vi "Create New File.vi"(8 "error in (no error)":errorcluster, 11 "file handler in":refnum<class "File Handler.lvclass">) -> (0 "error out":errorcluster, 3 "file handler out":refnum<class "File Handler.lvclass">)   [LabVIEW 2018, in "GLog.lvlib" / "File Handler.lvclass"]
uses:
  File Handler.lvclass
  File Handler.lvclass/File Handler.ctl
  Send Update Event.vi
  RolloverTrigger/RolloverTrigger.lvclass
panel:
  # "Connector Pane"
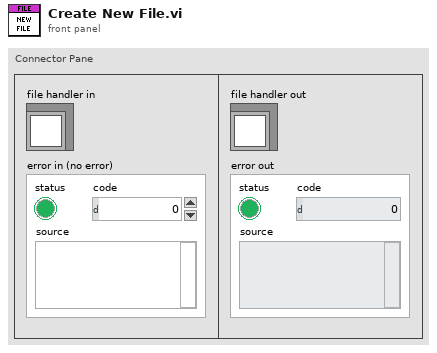
[diagram p1: front panel]
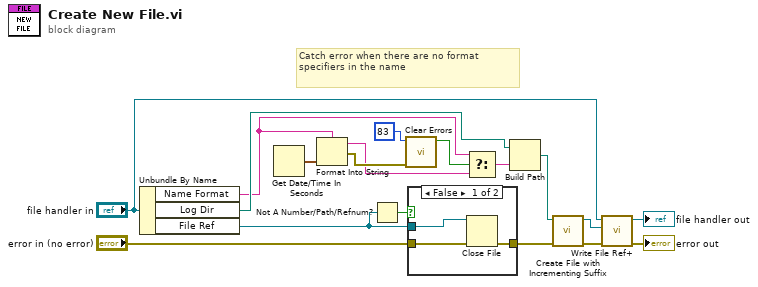
[diagram p0: block diagram]
diagram:
  # "Catch error when there are no format specifiers in the name"
  n1 = Unbundle By Name("file handler in") -> ("Name Format"=w3:string, "Log Dir"=w17:path, "File Ref"=w13:refnum<file>)
  n2 = Get Date/Time In Seconds() -> (seconds since 1Jan1904=w18:timestamp)
  n3 = Format Into String(format string=w3, w18) -> (resulting string=w2:string, error out=w6:errorcluster)  [unwired: 2 in]
  n4 = Not A Number/Path/Refnum?(number/path/refnum=w13) -> (NaN/Path/Refnum?=w12:bool)
  n5 = call <vilib>:"Clear Errors.vi"("error in (no error)"=w6, "specific error code to clear (0: all)"=83) -> ("specific error cleared?"=w4:bool)  [unwired: 4 in, 1 out]
  n6 = case shown="False" w12 {
    tunnel: "error in (no error)" -> [w21 w22]
    tunnel: [w20 w22] -> w14
    tunnel: w13 -> [w19 _]
    frame False {
      n7 = Close File(refnum=w19, error in=w21) -> (error out=w20:errorcluster)  [unwired: 1 out]
    }
    frame True {
    }
  }
  n8 = Select(t=w3, s=w4, f=w2) -> (s? t:f=w1:string)
  n9 = Build Path(base path=w17, name or relative path=w1) -> (appended path=w16:path)
  n10 = call <vilib>:"Create File with Incrementing Suffix.vi"("error in (no error)"=w14, "file path"=w16) -> ("error out"=w8:errorcluster, "refnum out"=w11:refnum<file>)  [unwired: 7 in, 1 out]
  n11 = call "Write File Ref+.vi"("error in (no error)"=w8, "File Ref"=w11, "File Handler in"="file handler in") -> ("error out"=→"error out":errorcluster, "File Handler out"=→"file handler out":refnum<class "File Handler.lvclass">)  [unwired: 7 in]
